vi "Failure.vi"(11 "Node In":refnum<class "bt_Node.lvclass">) -> (3 "Node":refnum<class "bt_Node.lvclass">)   [LabVIEW 2021, in "BT.lvlib"]
uses:
  BT.lvlib
  Support/Nodes/Decorators/Failure/bt_Failure.lvclass
  C:/Users/Tim/Documents/GitHub/LV_Behaviour_Tree/Source/Support/Nodes/Decorators/abs_Decorator/abs_Decorator.lvclass
  C:/Users/Tim/Documents/GitHub/LV_Behaviour_Tree/Source/Support/Nodes/abs_Node/bt_Node.lvclass
  C:/Users/Tim/Documents/GitHub/LV_Behaviour_Tree/Source/Support/Nodes/Decorators/Failure/bt_Failure.lvclass
  Support/Nodes/abs_Node/bt_Node.lvclass
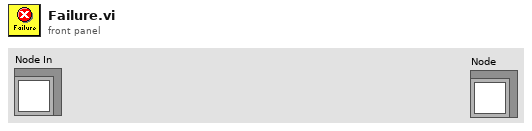
[diagram p1: front panel]
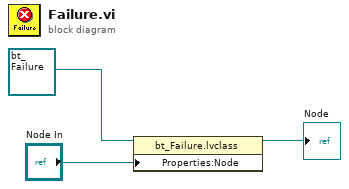
[diagram p0: block diagram]
diagram:
  n1 = property class="bt_Failure.lvclass"(reference=refnum<class "bt_Failure.lvclass"> refnum ("BT.lvlib:Failure.lvclass"), "Properties:Node"="Node In") -> (reference out=→"Node":refnum<class "bt_Failure.lvclass">)  [unwired: 1 in, 1 out]
